vi "W32B Build Wrapper.vi"(0 "template path":path, 1 "run in UI thread?":bool, 5 "target path":path, 7 "CLFN":T2, 9 "links":T1(array[cluster]), 11 "error in":errorcluster) -> (4 "wrapper path":path, 15 "error out":errorcluster)   [LabVIEW 2020]
doc: "Builds one Win32 wrapper VI by scripting. Opens the template VI and saves it as target path (the template file is not changed), resolves every link endpoint - a front-panel terminal by label, or the first input or output terminal of a node by class name, removing the template's placeholder wire at a node OUTPUT - then places a Call Library Function Node configured from CLFN (in LabVIEW's UI thread when run in UI thread? is TRUE, else in any thread) and wires each link's CLFN terminal to its endpoint, cleans up its block diagram, saves and closes the VI. CLFN terminal indices: 2 error in, 3 error out, 5 return value out, then input/output pairs from 6 per parameter."
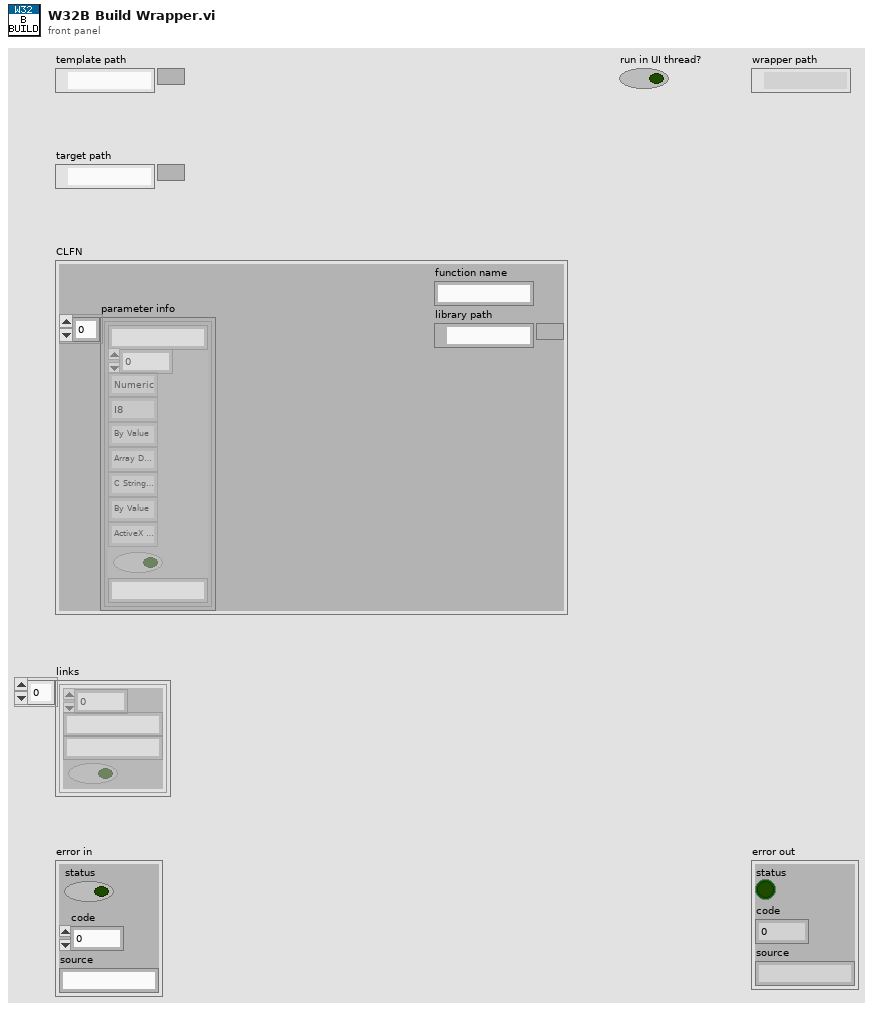
[diagram p1: front panel]
types:
  T1 = cluster{"CLFN terminal":i32, "control label":string, "node class":string, "node source?":bool}[]
  T2 = cluster{"function name":string, "library path":path, "parameter info":cluster{"Parameter Name":string, "Num Dimensions":i32, "Parameter Type":enum16{"Numeric", "Array", "String", "Waveform", "Digital Waveform", "Digital Table", "ActiveX", "Any", "Instance Data Pointer", "Void"}, "Numeric Type":enum16{"I8", "I16", "I32", "I64", "U8", "U16", "U32", "U64", "SGL", "DBL", "PTR INT", "PTR UINT"}, "Param Passing":enum16{"By Value", "Pointer To Value"}, "Array Passing":enum16{"Array Data Pointer", "Array Handle", "Array Handle Pointer"}, "String Passing":enum16{"C String Pointer", "Pascal String Pointer", "String Handle", "String Handle Pointer"}, "Adapt Format":enum16{"By Value", "Pointer To Value"}, "ActiveX Types":enum16{"ActiveX Variant Pointer", "IDispatch* Pointer", "IUnknown* Pointer"}, "Const (unused)":bool, "Minimum Size":string}[]}
  T3 = cluster{"Parameter Name":string, "Num Dimensions":i32, "Parameter Type":enum16{"Numeric", "Array", "String", "Waveform", "Digital Waveform", "Digital Table", "ActiveX", "Any", "Instance Data Pointer", "Void"}, "Numeric Type":enum16{"I8", "I16", "I32", "I64", "U8", "U16", "U32", "U64", "SGL", "DBL", "PTR INT", "PTR UINT"}, "Param Passing":enum16{"By Value", "Pointer To Value"}, "Array Passing":enum16{"Array Data Pointer", "Array Handle", "Array Handle Pointer"}, "String Passing":enum16{"C String Pointer", "Pascal String Pointer", "String Handle", "String Handle Pointer"}, "Adapt Format":enum16{"By Value", "Pointer To Value"}, "ActiveX Types":enum16{"ActiveX Variant Pointer", "IDispatch* Pointer", "IUnknown* Pointer"}, "Const (unused)":bool, "Minimum Size":string}[]
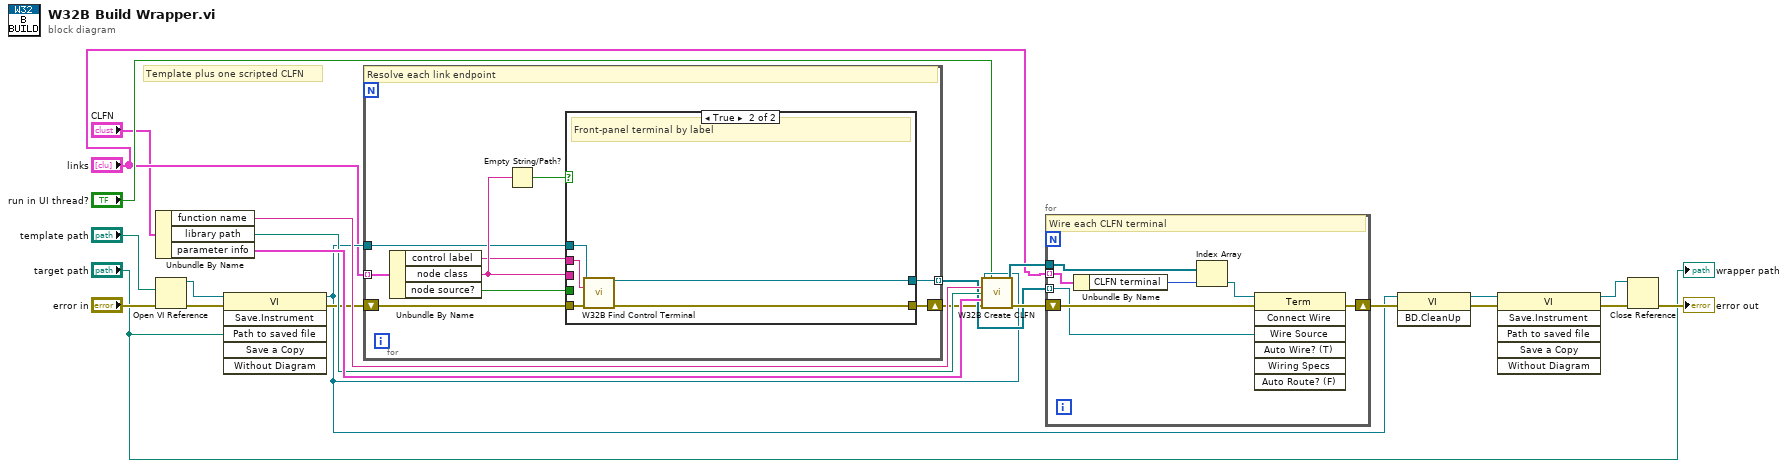
[diagram p0: block diagram]
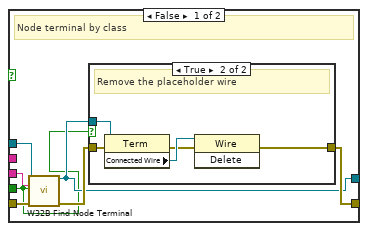
[diagram p2: hidden frame]
diagram:
  # "Template plus one scripted CLFN"
  n1 = Unbundle By Name("CLFN") -> ("function name"=w14:string, "library path"=w15:path, "parameter info"=w16:T3)
  n2 = Open VI Reference(vi path="template path", error in (no error)="error in") -> (vi reference=w8:refnum<vi>, error out=w9:errorcluster)  [unwired: 4 in]
  n3 = invoke class="VI" method="Save.Instrument"(reference=w8, error in=w9, "Path to saved file"="target path") -> (reference out=w10:refnum<vi>, error out=w11:errorcluster)  [unwired: 3 in, 4 out]
  n4 = for {
    tunnel: "links" -> [w24] mode=indexing
    tunnel: w10 -> [w25]
    shift-right: [w27] -> w12
    shift-left: w11 -> [w26]
    tunnel: [w32] -> w13 mode=indexing
    # "Resolve each link endpoint"
    n5 = Unbundle By Name(w24) -> ("control label"=w28:string, "node class"=w29:string, "node source?"=w30:bool)
    n6 = Empty String/Path?(string/path=w29) -> (empty?=w31:bool)
    n7 = case shown="True" w31 {
      tunnel: w28 -> [_ w47]
      tunnel: w29 -> [w34 _]
      tunnel: w30 -> [w35 _]
      tunnel: w25 -> [w33 w46]
      tunnel: w26 -> [w36 w48]
      tunnel: [w37 w49] -> w32
      tunnel: [w39 w50] -> w27
      frame False {
        # "Node terminal by class"
        n8 = call "W32B Find Node Terminal.vi"("VI reference"=w33, "node class"=w34, "source?"=w35, "error in"=w36) -> ("terminal"=w37:refnum<vi>, "error out"=w38:errorcluster)  [unwired: 10 in]
        n9 = case shown="True" w35 {
          tunnel: w37 -> [_ w41]
          tunnel: w38 -> [w40 w42]
          tunnel: [w40 w45] -> w39
          frame False {
          }
          frame True {
            # "Remove the placeholder wire"
            n10 = property class="Term"(reference=w41, error in=w42) -> (error out=w43:errorcluster, "Connected Wire"=w44:refnum<vi>)  [unwired: 1 out]
            n11 = invoke on="Invoke Node" class="Wire" method="Delete"(reference=w44, error in=w43) -> (error out=w45:errorcluster)  [unwired: 1 in, 2 out]
          }
        }
      }
      frame True {
        # "Front-panel terminal by label"
        n12 = call "W32B Find Control Terminal.vi"("VI reference"=w46, "label"=w47, "error in"=w48) -> ("terminal"=w49:refnum<vi>, "error out"=w50:errorcluster)  [unwired: 11 in]
      }
    }
  }
  n13 = call "W32B Create CLFN.vi"("VI reference"=w10, "run in UI thread?"="run in UI thread?", "function name"=w14, "library path"=w15, "parameter info"=w16, "error in"=w12) -> ("CLFN terminals"=w17:refnum<vi>[], "error out"=w18:errorcluster)  [unwired: 8 in]
  n14 = for {
    tunnel: "links" -> [w51] mode=indexing
    tunnel: w17 -> [w53]
    shift-right: [w55] -> w19
    shift-left: w18 -> [w54]
    tunnel: w13 -> [w52] mode=indexing
    # "Wire each CLFN terminal"
    n15 = Unbundle By Name(w51) -> ("CLFN terminal"=w56:i32)
    n16 = Index Array(array=w53, index=w56) -> (element=w57:refnum<vi>)
    n17 = invoke class="Term" method="Connect Wire"(reference=w57, error in=w54, "Wire Source"=w52) -> (error out=w55:errorcluster)  [unwired: 4 in, 6 out]
  }
  n18 = invoke class="VI" method="BD.CleanUp"(reference=w10, error in=w19) -> (reference out=w20:refnum<vi>, error out=w21:errorcluster)  [unwired: 1 in, 1 out]
  n19 = invoke class="VI" method="Save.Instrument"(reference=w20, error in=w21) -> (reference out=w22:refnum<vi>, error out=w23:errorcluster)  [unwired: 4 in, 4 out]
  n20 = Close Reference(reference=w22, error in (no error)=w23) -> (error out=→"error out":errorcluster)
  "wrapper path" <- "target path"
